vi "Smoothing++.vi"(9 "+/- Point":i32=3, 10 "Y in":dbl[](array[numeric])) -> (2 "Y out":dbl[](array[numeric]))   [LabVIEW 2018]
uses:
  <vilib>/Analysis/baseanly.llb/Mean (DBL).vi
  <vilib>/Analysis/NI_AALBase.lvlib
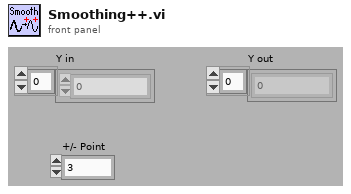
[diagram p1: front panel]
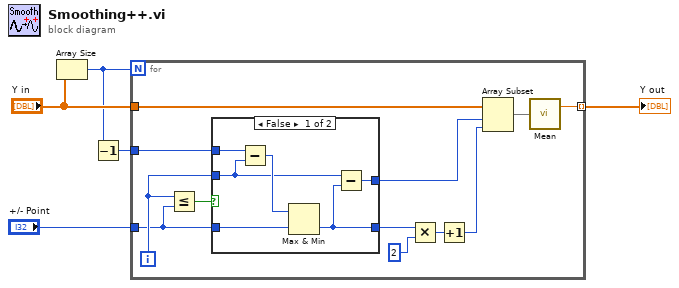
[diagram p0: block diagram]
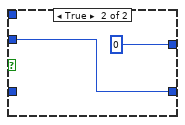
[diagram p2: hidden frame]
diagram:
  n1 = Array Size(array="Y in") -> (size(s)=w2:i32)
  n2 = Decrement(x=w2) -> (x-1=w1:i32)
  n3 = for {
    N: w2 -> [_]
    tunnel: "Y in" -> [w17]
    tunnel: "+/- Point" -> [w13]
    tunnel: [w7] -> w4 mode=indexing
    tunnel: w1 -> [w6]
    i -> [w14]
    n4 = Less Or Equal?(x=w14, y=w13) -> (x <= y?=w16:bool)
    n5 = case shown="False" w16 {
      tunnel: w14 -> [w18 w24]
      tunnel: [w23 0] -> w15
      tunnel: [w19 w24] -> w10
      tunnel: w13 -> [w21 _]
      tunnel: w6 -> [w22 _]
      frame False {
        n6 = Subtract(x=w22, y=w18) -> (x-y=w20:i32)
        n7 = Max & Min(x=w20, y=w21) -> (min(x,y)=w19:i32)  [unwired: 1 out]
        n8 = Subtract(x=w18, y=w19) -> (x-y=w23:i32)
      }
      frame True {
      }
    }
    n9 = Multiply(x=w10, y=2) -> (x*y=w12:i32)
    n10 = Increment(x=w12) -> (x+1=w9:i32)
    n11 = Array Subset(array=w17, index=w15, length=w9) -> (w8:dbl[])
    n12 = call-poly <vilib>:"Mean.vi"("X"=w8) -> ("mean"=w7:dbl)  [unwired: 1 out]
  }
  "Y out" <- w4
